vi "VIH Platform - Windows - Explore Folder.vi"(6 "cmd (run)":enum16{"run", "check"}(ring), 8 "error in":errorcluster, 11 "exe/doc/dir path":path) -> (0 "error out":errorcluster)   [LabVIEW 2014]
doc: "::: VI Helpeks :::\nCopyright (c) 2000-2026 Konstantin Shifershteyn. All rights reserved."
panel:
  # "VI Helpeks\nCopyright (c) 2012-2026 Konstantin Shifershteyn"
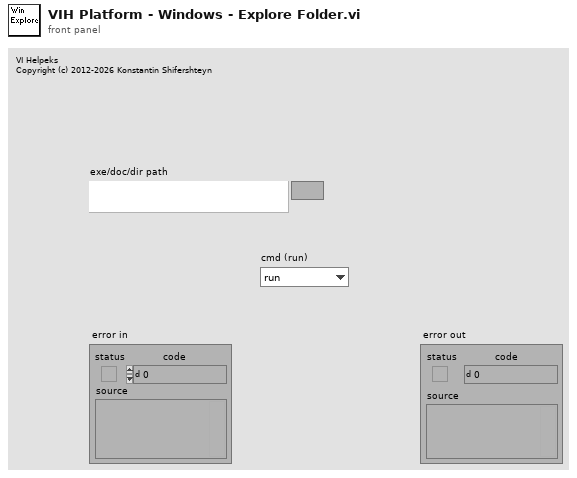
[diagram p1: front panel]
types:
  T1 = enum32{"edit", "explore", "find", "open", "print"}
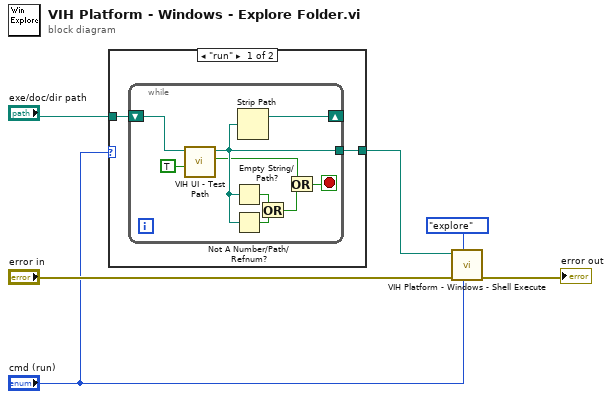
[diagram p0: block diagram]
diagram:
  n1 = case shown="\"run\"" "cmd (run)" {
    tunnel: "exe/doc/dir path" -> [w8 w18]
    tunnel: [w7 w18] -> w1
    frame "run" {
      n2 = while {
        tunnel: [w12] -> w7
        shift-right: [w15] -> _
        shift-left: w8 -> [w17]
        stop <- w9 stop-if-true
        n3 = call "VIH UI - Test Path.vi"("Folder (F)"=TRUE, "Path"=w17) -> ("Good Path"=w11:bool, "dup Path"=w12:path)  [unwired: 6 in, 2 out]
        n4 = Empty String/Path?(string/path=w12) -> (empty?=w14:bool)
        n5 = Not A Number/Path/Refnum?(number/path/refnum=w12) -> (NaN/Path/Refnum?=w13:bool)
        n6 = Strip Path(path=w12) -> (stripped path=w15:path)  [unwired: 1 out]
        n7 = Or(x=w14, y=w13) -> (x .or. y?=w10:bool)
        n8 = Or(x=w11, y=w10) -> (x .or. y?=w9:bool)
      }
    }
    frame "check" {
    }
  }
  n9 = call "VIH Platform - Windows - Shell Execute.vi"("cmd (run)"="cmd (run)", "Shell action (open)"=T1."explore", "error in"="error in", "exe/doc/dir path"=w1) -> ("error out"=→"error out":errorcluster)  [unwired: 7 in]
